vi "M-686 Stage Engine.vi"(0 "Notifier Name":string, 11 "COM Port":string[](array[string])) -> ()   [LabVIEW 2016]
uses:
  Stages Controls/Stage Notifier Element.ctl
  Stages Controls/Stage Actions.ctl
  Stages Controls/Stage Status.ctl
  <vilib>/Instr/_visa.llb/VISA Configure Serial Port (Instr).vi
panel:
  in  "Servo On/Off":bool
  in  "Quit":bool
  in  "Halt":bool
  in  "Home":bool
  in  "Get Position":bool
  in  "Y Position (µm)":dbl format="%#_4g"
  in  "X Position (µm)":dbl format="%#_4g"
  in  "XY Step Size (µm)":dbl format="%#_4g"
  in  "Up":bool
  in  "Down":bool
  in  "Left":bool
  in  "Right":bool
  in  "ReInitialize":bool
  in  "Error":bool
  # "(1) COM Port\n(2) Axis Name\n(3) Axis Name"
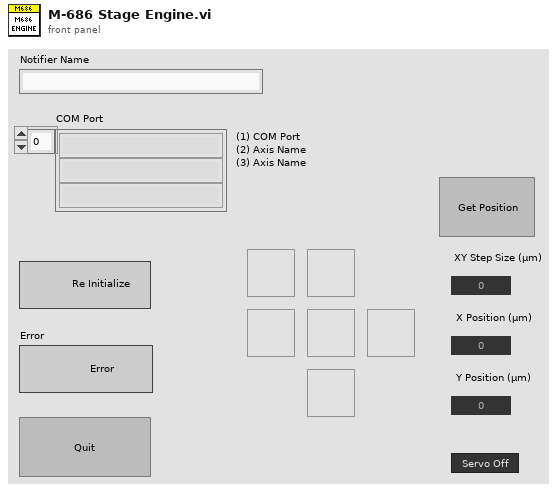
[diagram p1: front panel]
types:
  T1 = typedef "Stage Notifier Element.ctl" = cluster{"Action":T2, "Axis":bool[], "Setpoint":dbl[], "Velocity":dbl, "Cmd Recvd?":bool, "Position":dbl[], "Status":T3, "Misc":variant, "Servo On?":bool}
  T2 = typedef "Stage Actions.ctl" = enum16{"Get Position", "SERVO OFF", "SERVO ON", "SERVO ON/OFF", "MVR", "MOVE", "HALT", "ONTARGET", "ERROR", "REFERENCE", "INIT", "VELOCITY", "STATUS", "EXIT", "HOME", "ZEROPOS", "NANOPOS", "ANALOG", "QUIT"}
  T3 = typedef "Stage Status.ctl" = enum16{"Error", "Abort", "Busy", "On Target"}
  T4 = enum32{"Invalid", "Standard", "Closed", "Hidden", "Minimized", "Maximized"}
  T5 = enum8{"Enabled", "Disabled", "Disabled and Grayed Out"}
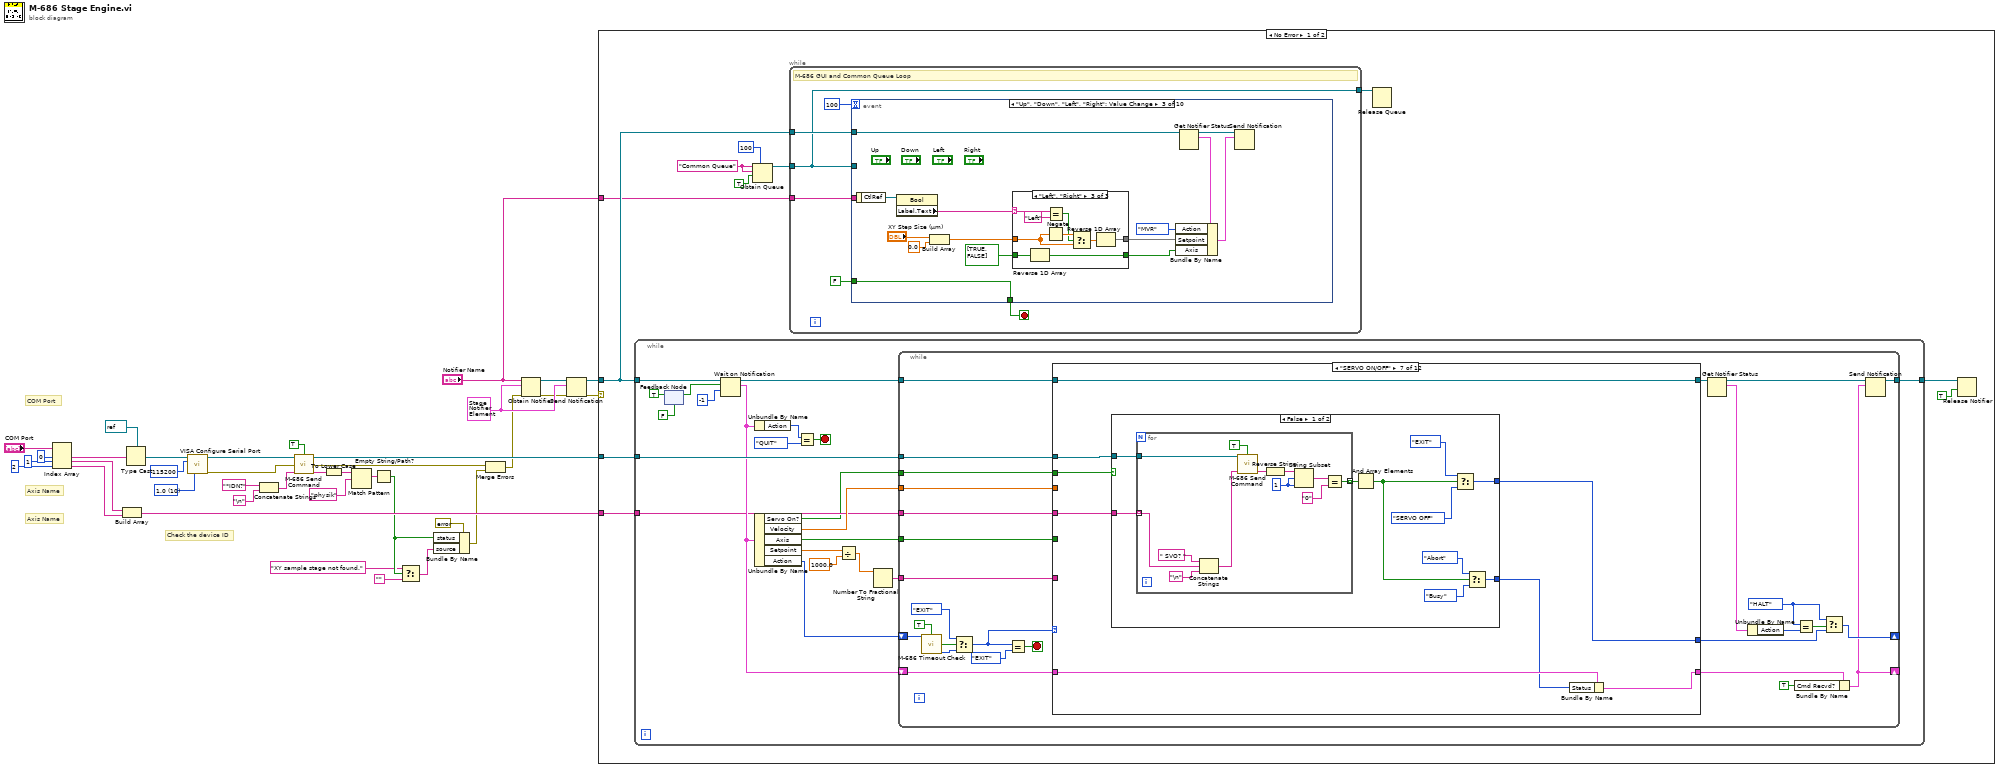
[diagram p0: block diagram]
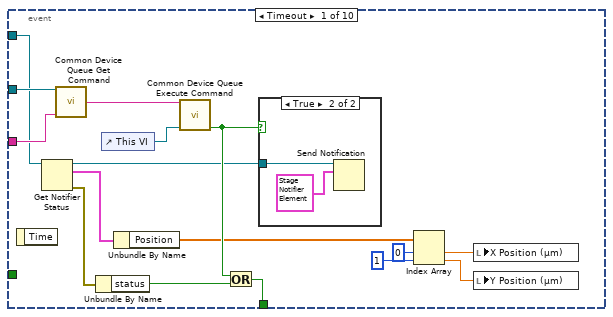
[diagram p2: hidden frame]
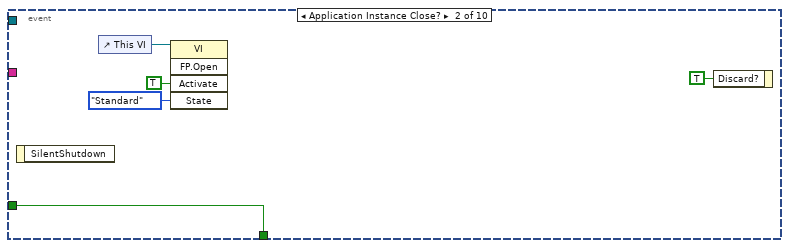
[diagram p4: hidden frame]
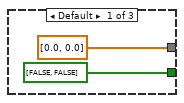
[diagram p5: hidden frame]
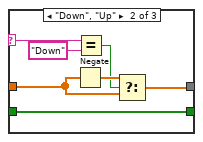
[diagram p6: hidden frame]
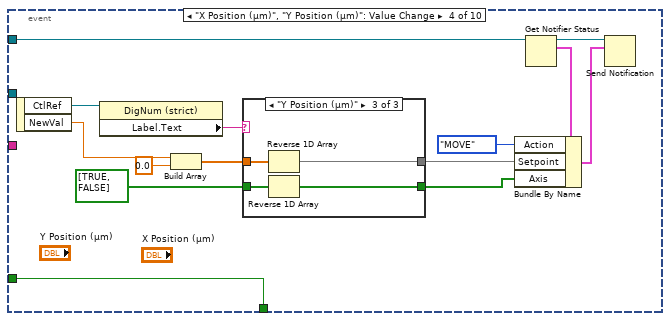
[diagram p7: hidden frame]
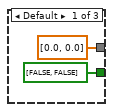
[diagram p8: hidden frame]
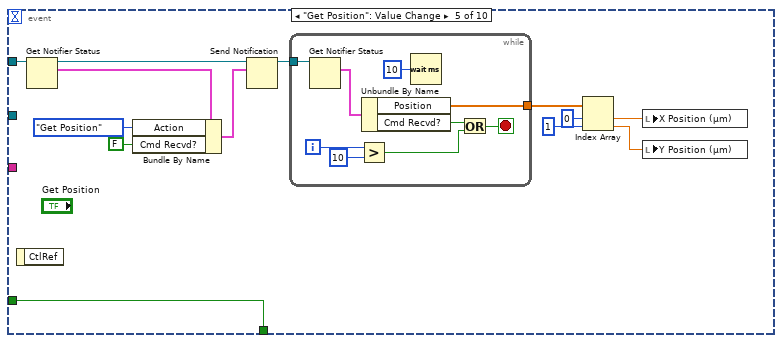
[diagram p10: hidden frame]
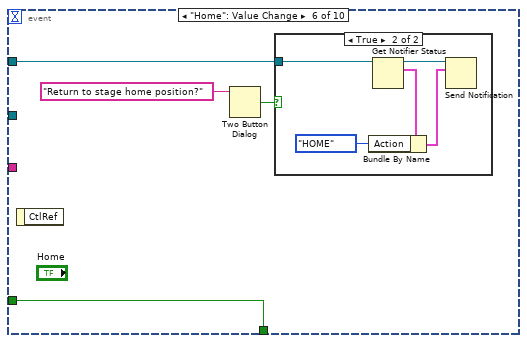
[diagram p11: hidden frame]
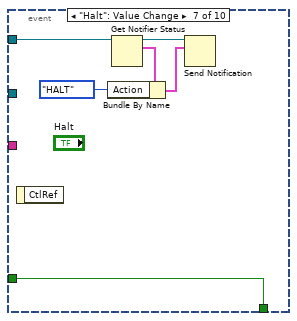
[diagram p13: hidden frame]
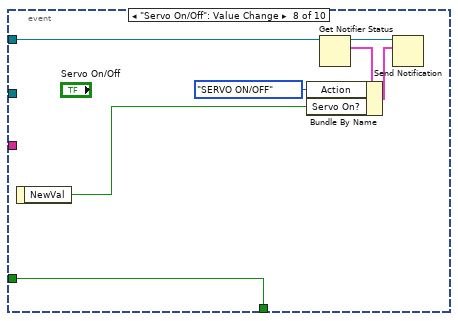
[diagram p14: hidden frame]
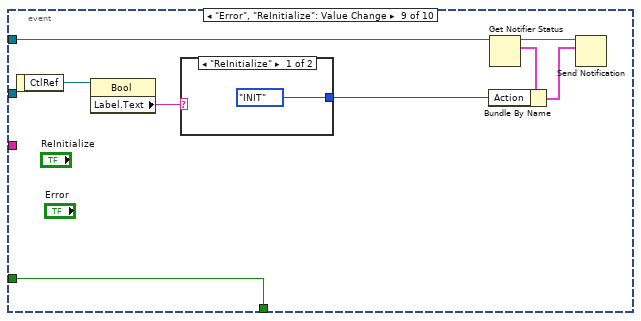
[diagram p15: hidden frame]
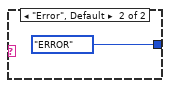
[diagram p16: hidden frame]
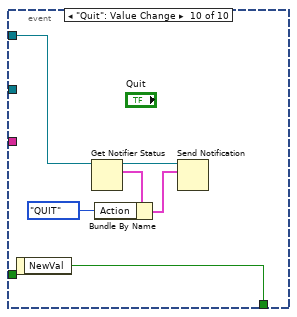
[diagram p17: hidden frame]
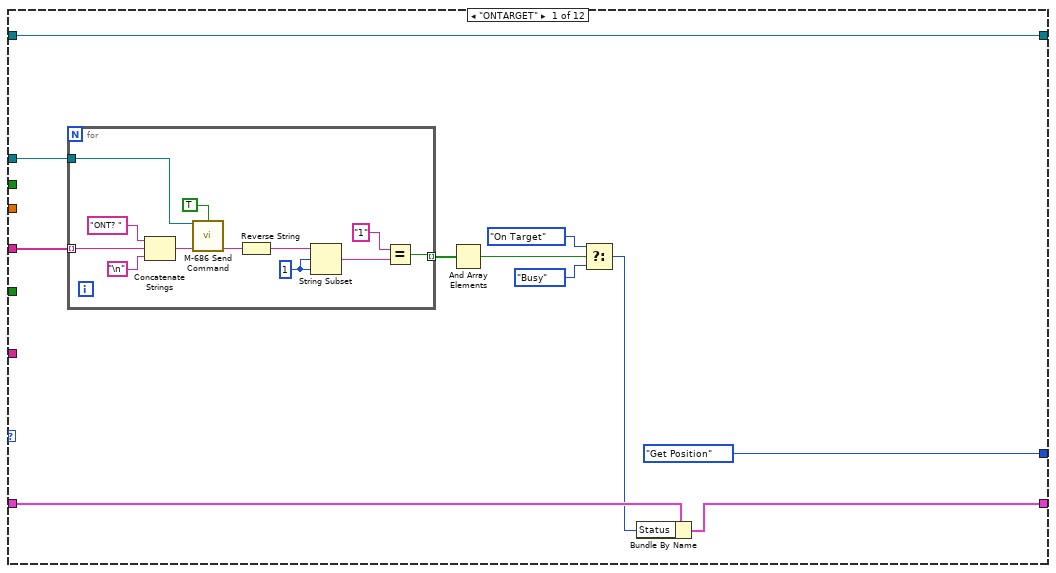
[diagram p18: hidden frame]
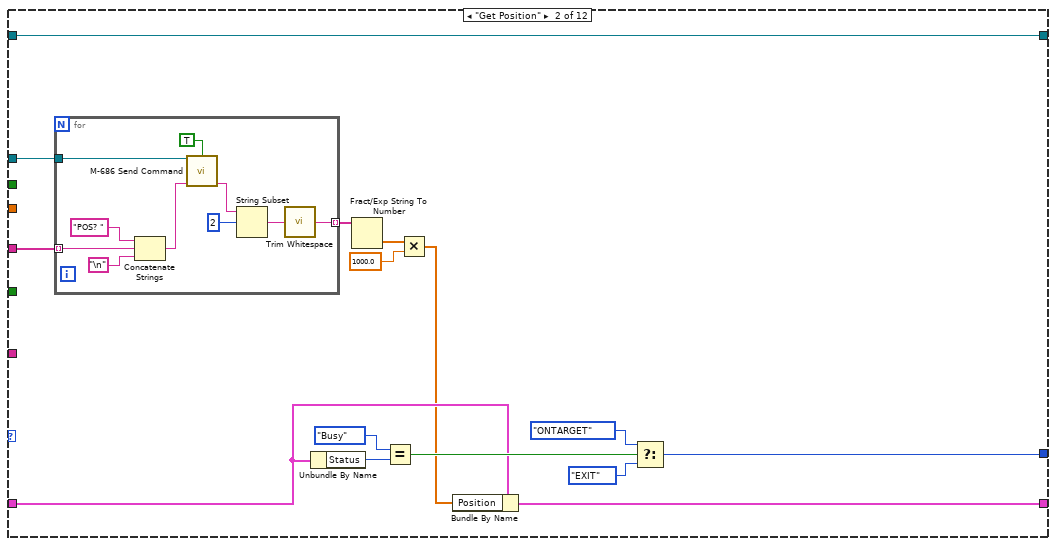
[diagram p19: hidden frame]
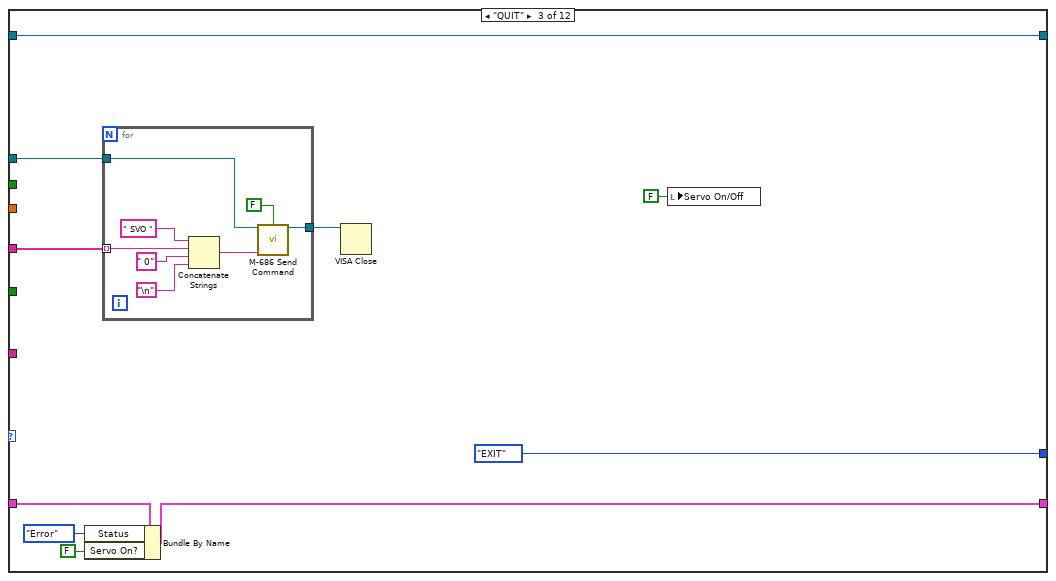
[diagram p20: hidden frame]
diagram:
  w21 = u16 10 items=["1.0"=10, "1.5"=15, "2.0"=20] ("stop bits (10: 1 bit)")
  w32 = T1 {"Action"=enum."INIT", "Axis"=[], "Setpoint"=[], "Velocity"=0.5, "Cmd Recvd?"=FALSE, "Position"=[], "Status"=enum."Busy", "Misc"=variant, "Servo On?"=FALSE} ("Stage Status")
  # "Check the device ID"
  # "Axis Name"
  # "Axis Name"
  # "COM Port"
  n1 = Index Array(array="COM Port", index #1=0 ("index"), index #2=1 ("index"), index #3=2 ("index")) -> (element #1=w36:string, element #2=w25:string, element #3=w24:string)
  n2 = Build Array(w25, w24) -> (w23:string[])
  n3 = Type Cast(type=refnum<visa-resource-name> refnum ("reference out"), x=w36) -> (*(type *) &x=w20:refnum<visa-resource-name>)
  n4 = call-poly "VISA Configure Serial Port"("VISA resource name"=w20, "baud rate (9600)"=u32 115200, "stop bits (10: 1 bit)"=w21) -> ("VISA resource name out"=w19:refnum<visa-resource-name>, "error out"=w18:errorcluster)  [unwired: 11 in]
  n5 = Concatenate Strings("*IDN?" ("string"), "\n") -> (w16:string)
  n6 = call "M-686 Send Command.vi"("VISA Ref"=w19, "Wait for Reply?"=TRUE, "Error In"=w18, "Command"=w16) -> ("VISA Ref Out"=w17:refnum<visa-resource-name>, "Error Out"=w7:errorcluster, "Response"=w9:string)  [unwired: 9 in]
  n7 = To Lower Case(string=w9) -> (all lower case string=w12:string)
  n8 = Match Pattern(string=w12, regular expression="physik" ("string")) -> (match substring=w11:string)  [unwired: 1 in, 3 out]
  n9 = Empty String/Path?(string/path=w11) -> (empty?=w4:bool)
  n10 = Select(t="XY sample stage not found." ("string"), s=w4, f="") -> (s? t:f=w3:string)
  n11 = Bundle By Name(cluster=errorcluster {"status"=FALSE, "code"=0, "source"=""} ("Error Out"), "status"=w4, "source"=w3) -> (w5:errorcluster)
  n12 = Merge Errors(w7, w5) -> (w6:errorcluster)
  n13 = Obtain Notifier(name (unnamed)="Notifier Name", notification data type=w32, error in (no error)=w6) -> (notifier out=w33:refnum<notifier>, error out=w31:errorcluster)  [unwired: 1 in, 1 out]
  n14 = Send Notification(notification=w32, notifier=w33, error in (no error)=w31) -> (notifier out=w30:refnum<notifier>, error out=w29:errorcluster)
  n15 = case shown="No Error" w29 {
    selector: w29 -> [_ w573]
    tunnel: w17 -> [w48 w574]
    tunnel: w30 -> [w41 w575]
    tunnel: "Notifier Name" -> [w40 _]
    tunnel: w23 -> [w38 _]
    frame No Error {
      w44 = "Common Queue" ("Unique Notifier Name")
      n16 = while {
        tunnel: w41 -> [w210]
        tunnel: w48 -> [w202]
        tunnel: [w199] -> w47
        tunnel: w38 -> [w195]
        stop <- w212 stop-if-true
        n17 = feedback-in #1(TRUE) -> ()
        n18 = feedback #1(FALSE) -> (w196:bool)
        n19 = Wait on Notification(notifier=w210, ignore previous (F)=w196, timeout in ms (-1)=-1) -> (notifier out=w201:refnum<notifier>, notification=w200:T1)  [unwired: 1 in, 2 out]
        n20 = Unbundle By Name(w200) -> ("Action"=w209:T2)
        n21 = Unbundle By Name(w200) -> ("Servo On?"=w192:bool, "Velocity"=w206:dbl, "Axis"=w205:bool[], "Setpoint"=w204:dbl[], "Action"=w194:T2)
        n22 = Equal?(x=w209, y=Stage_Actions."QUIT") -> (x = y?=w212:bool)
        n23 = Divide(x=w204, y=1000.0) -> (x/y=w193:dbl[])
        n24 = Number To Fractional String(number=w193) -> (F-format string=w207:string[])  [unwired: 3 in]
        n25 = while {
          tunnel: w195 -> [w240]
          shift-right: [w233] -> _
          shift-left: w194 -> [w230]
          tunnel: w205 -> [w237]
          tunnel: w206 -> [w236]
          tunnel: w207 -> [w238]
          shift-right: [w216] -> _
          shift-left: w200 -> [w235]
          tunnel: w202 -> [w239]
          tunnel: w201 -> [w215]
          tunnel: [w219] -> w199
          tunnel: w192 -> [w213]
          stop <- w231 stop-if-true
          w222 = Stage_Actions."HALT" ("Action")
          n26 = call "M-686 Timeout Check.vi"("Action"=w230, "User Input?"=TRUE) -> ("Timeout?"=w229:bool, "Action (Dup)"=w227:T2)  [unwired: 12 in]
          n27 = Select(t=Stage_Actions."EXIT" ("y"), s=w229, f=w227) -> (s? t:f=w226:T2)
          n28 = Equal?(x=w226, y=Stage_Actions."EXIT") -> (x = y?=w231:bool)
          n29 = case shown="\"SERVO ON/OFF\"" w226 {
            selector: w226 -> [_ _ _ _ _ _ _ _ _ _ _ w531]
            tunnel: w240 -> [w249 w277 w297 _ _ w345 w381 w434 w464 w482 w516 w543]
            tunnel: w239 -> [w251 w278 w298 _ w314 w336 w382 w435 w465 w481 w511 w537]
            tunnel: w238 -> [_ _ _ _ _ _ _ _ _ _ _ w534]
            tunnel: w237 -> [_ _ _ _ _ _ _ _ _ _ _ w525]
            tunnel: w236 -> [_ _ _ _ _ _ _ _ _ _ _ w542]
            tunnel: [Stage_Actions."Get Position" ("Action") w275 Stage_Actions."EXIT" ("Action") Stage_Actions."EXIT" ("Action") w324 w344 w380 w433 Stage_Actions."EXIT" ("Action") w477 Stage_Actions."EXIT" ("Action") Stage_Actions."ONTARGET" ("Action")] -> w234
            tunnel: w235 -> [w244 w272 w295 w309 w322 w346 w378 w431 w460 w475 w513 w539]
            tunnel: [w242 w270 w293 w309 w323 w347 w377 w429 w459 w474 w512 w538] -> w218
            tunnel: w215 -> [w241 w264 w289 w307 w310 w330 w379 w432 w462 w473 w510 w523]
            tunnel: [w241 w264 w289 w307 w310 w330 w379 w432 w462 w473 w510 w523] -> w214
            tunnel: w213 -> [_ _ _ _ _ _ w383 _ _ _ _ _]
            frame "ONTARGET" {
              n30 = for {
                tunnel: [w261] -> w250 mode=indexing
                tunnel: w249 -> [w256] mode=indexing
                tunnel: w251 -> [w253]
                w257 = 1 ("length (rest)")
                n31 = Concatenate Strings("ONT? " ("string"), w256, "\n") -> (w255:string)
                n32 = call "M-686 Send Command.vi"("VISA Ref"=w253, "Wait for Reply?"=TRUE, "Command"=w255) -> ("Response"=w252:string)  [unwired: 10 in, 2 out]
                n33 = Reverse String(1:w252) -> (0:w258:string)
                n34 = String Subset(string=w258, offset (0)=w257, length (rest)=w257) -> (substring=w263:string)
                n35 = Equal?(x="1", y=w263) -> (x = y?=w261:bool)
              }
              n36 = And Array Elements(Boolean array=w250) -> (logical AND=w245:bool)
              n37 = Select(t=Stage_Status."On Target" ("Status"), s=w245, f=Stage_Status."Busy" ("Status")) -> (s? t:f=w243:T3)
              n38 = Bundle By Name(cluster=w244, "Status"=w243) -> (w242:T1)
            }
            frame "Get Position" {
              n39 = for {
                tunnel: [w288] -> w276 mode=indexing
                tunnel: w277 -> [w283] mode=indexing
                tunnel: w278 -> [w282]
                n40 = Concatenate Strings("POS? " ("string"), w283, "\n") -> (w281:string)
                n41 = call "M-686 Send Command.vi"("VISA Ref"=w282, "Wait for Reply?"=TRUE, "Command"=w281) -> ("Response"=w279:string)  [unwired: 10 in, 2 out]
                n42 = String Subset(string=w279, offset (0)=2) -> (substring=w284:string)  [unwired: 1 in]
                n43 = call <vilib>:"Trim Whitespace.vi"("string"=w284) -> ("trimmed string"=w288:string)  [unwired: 1 in]
              }
              n44 = Unbundle By Name(w272) -> ("Status"=w271:T3)
              n45 = Fract/Exp String To Number(string=w276) -> (number=w269:dbl[])  [unwired: 3 in, 1 out]
              n46 = Equal?(x=Stage_Status."Busy", y=w271) -> (x = y?=w273:bool)
              n47 = Multiply(x=w269, y=1000.0) -> (x*y=w266:dbl[])
              n48 = Bundle By Name(cluster=w272, "Position"=w266) -> (w270:T1)
              n49 = Select(t=Stage_Actions."ONTARGET" ("Action"), s=w273, f=Stage_Actions."EXIT" ("Action")) -> (s? t:f=w275:T2)
            }
            frame "QUIT" {
              n50 = Bundle By Name(cluster=w295, "Status"=Stage_Status."Error", "Servo On?"=FALSE) -> (w293:T1)
              n51 = for {
                tunnel: w298 -> [w300]
                tunnel: w297 -> [w303] mode=indexing
                tunnel: [w299] -> w292
                n52 = Concatenate Strings(" SVO " ("string"), w303, " 0" ("string"), "\n") -> (w302:string)
                n53 = call "M-686 Send Command.vi"("VISA Ref"=w300, "Wait for Reply?"=FALSE, "Command"=w302) -> ("VISA Ref Out"=w299:refnum<visa-resource-name>)  [unwired: 10 in, 2 out]
              }
              n54 = VISA Close(VISA resource name=w292) -> ()  [unwired: 1 in, 1 out]
              n55 = local write "Servo On/Off"(FALSE ("Servo On/Off")) -> ()
            }
            frame "EXIT", Default {
            }
            frame "ERROR" {
              n56 = Concatenate Strings(" ERR?" ("string"), "\n") -> (w312:string)
              n57 = call "M-686 Send Command.vi"("VISA Ref"=w314, "Wait for Reply?"=TRUE, "Command"=w312) -> ("Response"=w311:string)  [unwired: 10 in, 2 out]
              n58 = Reverse String(1:w311) -> (0:w319:string)
              n59 = String Subset(string=w319, offset (0)=1) -> (substring=w321:string)  [unwired: 1 in]
              n60 = Equal?(x=w321, y="0") -> (x = y?=w315:bool)
              n61 = Select(t=Stage_Status."Busy" ("Status"), s=w315, f=Stage_Status."Error" ("Status")) -> (s? t:f=w327:T3)
              n62 = Bundle By Name(cluster=w322, "Status"=w327) -> (w323:T1)
              n63 = Select(t=Stage_Actions."ONTARGET" ("Action"), s=w315, f=Stage_Actions."ERROR") -> (s? t:f=w324:T2)
            }
            frame "INIT" {
              n64 = Concatenate Strings(" ERR?" ("string"), "\n") -> (w333:string)
              n65 = call "M-686 Send Command.vi"("VISA Ref"=w336, "Wait for Reply?"=TRUE, "Command"=w333) -> ("VISA Ref Out"=w335:refnum<visa-resource-name>, "Response"=w332:string)  [unwired: 10 in, 1 out]
              n66 = Reverse String(1:w332) -> (0:w342:string)
              n67 = String Subset(string=w342, offset (0)=1) -> (substring=w340:string)  [unwired: 1 in]
              n68 = Equal?(x=w340, y="0") -> (x = y?=w337:bool)
              n69 = case shown="True" w337 {
                tunnel: w345 -> [_ w357]
                tunnel: [Stage_Actions."INIT" ("Action") w355] -> w344
                tunnel: w335 -> [_ w353]
                tunnel: [w349 w351] -> w331
                frame False {
                  w349 = FALSE
                  n70 = local write "Servo On/Off"(w349) -> ()
                }
                frame True {
                  n71 = for {
                    tunnel: w357 -> [w371] mode=indexing
                    tunnel: w353 -> [w364]
                    tunnel: [w366] -> w352 mode=indexing
                    w370 = 1 ("length (rest)")
                    n72 = Concatenate Strings(" SVO " ("string"), w371, " 1" ("string"), "\n") -> (w363:string)
                    n73 = Concatenate Strings(" SVO? " ("string"), w371, "\n") -> (w360:string)
                    n74 = call "M-686 Send Command.vi"("VISA Ref"=w364, "Wait for Reply?"=FALSE, "Command"=w363) -> ("VISA Ref Out"=w361:refnum<visa-resource-name>)  [unwired: 10 in, 2 out]
                    n75 = call "M-686 Send Command.vi"("VISA Ref"=w361, "Wait for Reply?"=TRUE, "Command"=w360) -> ("Response"=w358:string)  [unwired: 10 in, 2 out]
                    n76 = Reverse String(1:w358) -> (0:w369:string)
                    n77 = String Subset(string=w369, offset (0)=w370, length (rest)=w370) -> (substring=w368:string)
                    n78 = Equal?(x=w368, y="1") -> (x = y?=w366:bool)
                  }
                  n79 = And Array Elements(Boolean array=w352) -> (logical AND=w351:bool)
                  n80 = local write "Servo On/Off"(w351) -> ()
                  n81 = Select(t=Stage_Actions."REFERENCE" ("Action"), s=w351, f=Stage_Actions."INIT" ("Action")) -> (s? t:f=w355:T2)
                }
              }
              n82 = Bundle By Name(cluster=w346, "Status"=Stage_Status."Busy", "Servo On?"=w331) -> (w347:T1)
            }
            frame "SERVO ON/OFF" {
              n83 = case shown="False" w383 {
                tunnel: w381 -> [w389 w415]
                tunnel: [w388 w410] -> w380
                tunnel: w382 -> [w390 w414]
                tunnel: [w384 w406] -> w376
                frame False {
                  n84 = for {
                    tunnel: w389 -> [w403] mode=indexing
                    tunnel: w390 -> [w394]
                    tunnel: [w398] -> w393 mode=indexing
                    w402 = 1 ("length (rest)")
                    n85 = Concatenate Strings(" SVO? " ("string"), w403, "\n") -> (w397:string)
                    n86 = call "M-686 Send Command.vi"("VISA Ref"=w394, "Wait for Reply?"=TRUE, "Command"=w397) -> ("Response"=w395:string)  [unwired: 10 in, 2 out]
                    n87 = Reverse String(1:w395) -> (0:w401:string)
                    n88 = String Subset(string=w401, offset (0)=w402, length (rest)=w402) -> (substring=w400:string)
                    n89 = Equal?(x=w400, y="0") -> (x = y?=w398:bool)
                  }
                  n90 = And Array Elements(Boolean array=w393) -> (logical AND=w385:bool)
                  n91 = Select(t=Stage_Actions."EXIT" ("Action"), s=w385, f=Stage_Actions."SERVO OFF") -> (s? t:f=w388:T2)
                  n92 = Select(t=Stage_Status."Abort", s=w385, f=Stage_Status."Busy" ("Status")) -> (s? t:f=w384:T3)
                }
                frame True {
                  n93 = for {
                    tunnel: w415 -> [w425] mode=indexing
                    tunnel: w414 -> [w416]
                    tunnel: [w420] -> w413 mode=indexing
                    w424 = 1 ("length (rest)")
                    n94 = Concatenate Strings(" SVO? " ("string"), w425, "\n") -> (w419:string)
                    n95 = call "M-686 Send Command.vi"("VISA Ref"=w416, "Wait for Reply?"=TRUE, "Command"=w419) -> ("Response"=w417:string)  [unwired: 10 in, 2 out]
                    n96 = Reverse String(1:w417) -> (0:w423:string)
                    n97 = String Subset(string=w423, offset (0)=w424, length (rest)=w424) -> (substring=w422:string)
                    n98 = Equal?(x=w422, y="1") -> (x = y?=w420:bool)
                  }
                  n99 = And Array Elements(Boolean array=w413) -> (logical AND=w409:bool)
                  n100 = Select(t=Stage_Actions."EXIT" ("Action"), s=w409, f=Stage_Actions."SERVO ON") -> (s? t:f=w410:T2)
                  n101 = Select(t=Stage_Status."On Target", s=w409, f=Stage_Status."Busy" ("Status")) -> (s? t:f=w406:T3)
                }
              }
              n102 = Bundle By Name(cluster=w378, "Status"=w376) -> (w377:T1)
            }
            frame "SERVO ON" {
              w428 = T5."Enabled" ("Disabled")
              n103 = for {
                tunnel: w434 -> [w453] mode=indexing
                tunnel: w435 -> [w446]
                tunnel: [w448] -> w436 mode=indexing
                w452 = 1 ("length (rest)")
                n104 = Concatenate Strings(" SVO " ("string"), w453, " 1" ("string"), "\n") -> (w445:string)
                n105 = Concatenate Strings(" SVO? " ("string"), w453, "\n") -> (w442:string)
                n106 = call "M-686 Send Command.vi"("VISA Ref"=w446, "Wait for Reply?"=FALSE, "Command"=w445) -> ("VISA Ref Out"=w443:refnum<visa-resource-name>)  [unwired: 10 in, 2 out]
                n107 = call "M-686 Send Command.vi"("VISA Ref"=w443, "Wait for Reply?"=TRUE, "Command"=w442) -> ("Response"=w440:string)  [unwired: 10 in, 2 out]
                n108 = Reverse String(1:w440) -> (0:w451:string)
                n109 = String Subset(string=w451, offset (0)=w452, length (rest)=w452) -> (substring=w450:string)
                n110 = Equal?(x=w450, y="1") -> (x = y?=w448:bool)
              }
              n111 = Bundle By Name(cluster=w431, "Status"=Stage_Status."Busy") -> (w429:T1)
              n112 = And Array Elements(Boolean array=w436) -> (logical AND=w437:bool)
              n113 = Select(t=Stage_Actions."Get Position" ("Action"), s=w437, f=Stage_Actions."SERVO ON" ("Action")) -> (s? t:f=w433:T2)
              n114 = property on="Down" class="Bool"("DisabledEnum"=w428) -> ()  [unwired: 2 in, 2 out]
              n115 = property on="Up" class="Bool"("DisabledEnum"=w428) -> ()  [unwired: 2 in, 2 out]
              n116 = property on="Y Position (µm)" class="DigNum (strict)"("DisabledEnum"=w428) -> ()  [unwired: 2 in, 2 out]
              n117 = property on="Right" class="Bool"("DisabledEnum"=w428) -> ()  [unwired: 2 in, 2 out]
              n118 = property on="Left" class="Bool"("DisabledEnum"=w428) -> ()  [unwired: 2 in, 2 out]
              n119 = property on="X Position (µm)" class="DigNum (strict)"("DisabledEnum"=w428) -> ()  [unwired: 2 in, 2 out]
            }
            frame "SERVO OFF" {
              w458 = T5."Disabled and Grayed Out" ("Disabled")
              n120 = for {
                tunnel: w465 -> [w466]
                tunnel: w464 -> [w469] mode=indexing
                n121 = Concatenate Strings(" SVO " ("string"), w469, " 0" ("string"), "\n") -> (w468:string)
                n122 = call "M-686 Send Command.vi"("VISA Ref"=w466, "Wait for Reply?"=FALSE, "Command"=w468) -> ()  [unwired: 10 in, 3 out]
              }
              n123 = Bundle By Name(cluster=w460, "Status"=Stage_Status."Abort") -> (w459:T1)
              n124 = property on="X Position (µm)" class="DigNum (strict)"("DisabledEnum"=w458) -> ()  [unwired: 2 in, 2 out]
              n125 = property on="Y Position (µm)" class="DigNum (strict)"("DisabledEnum"=w458) -> ()  [unwired: 2 in, 2 out]
              n126 = property on="Down" class="Bool"("DisabledEnum"=w458) -> ()  [unwired: 2 in, 2 out]
              n127 = property on="Right" class="Bool"("DisabledEnum"=w458) -> ()  [unwired: 2 in, 2 out]
              n128 = property on="Left" class="Bool"("DisabledEnum"=w458) -> ()  [unwired: 2 in, 2 out]
              n129 = property on="Up" class="Bool"("DisabledEnum"=w458) -> ()  [unwired: 2 in, 2 out]
            }
            frame "REFERENCE" {
              n130 = for {
                tunnel: w482 -> [w507] mode=indexing
                tunnel: w481 -> [w501]
                tunnel: [w500] -> w478
                tunnel: [w502] -> w480 mode=indexing
                w505 = 1 ("length (rest)")
                n131 = Concatenate Strings(" FRF? " ("string"), w507, "\n") -> (w499:string)
                n132 = call "M-686 Send Command.vi"("VISA Ref"=w501, "Wait for Reply?"=TRUE, "Command"=w499) -> ("VISA Ref Out"=w500:refnum<visa-resource-name>, "Response"=w498:string)  [unwired: 10 in, 1 out]
                n133 = Reverse String(1:w498) -> (0:w506:string)
                n134 = String Subset(string=w506, offset (0)=w505, length (rest)=w505) -> (substring=w503:string)
                n135 = Equal?(x=w503, y="1") -> (x = y?=w502:bool)
              }
              n136 = Bundle By Name(cluster=w475, "Status"=Stage_Status."Busy") -> (w474:T1)
              n137 = And Array Elements(Boolean array=w480) -> (logical AND=w479:bool)
              n138 = case shown="True" w479 {
                tunnel: w478 -> [w484 _]
                tunnel: [w483 Stage_Actions."ONTARGET" ("Action")] -> w477
                frame False {
                  n139 = Two Button Dialog(message="M686", 1:"Skip" ("F button name (\"Cancel\")"), 2:"Reference" ("T button name (\"OK\")")) -> (T button?=w488:bool)
                  n140 = case shown="True" w488 {
                    tunnel: [Stage_Actions."HALT" ("Action") Stage_Actions."ONTARGET" ("Action")] -> w483
                    tunnel: w484 -> [_ w492]
                    frame False {
                    }
                    frame True {
                      n141 = Concatenate Strings("FRF" ("string"), "\n") -> (w491:string)
                      n142 = call "M-686 Send Command.vi"("VISA Ref"=w492, "Wait for Reply?"=FALSE, "Command"=w491) -> ()  [unwired: 10 in, 3 out]
                    }
                  }
                }
                frame True {
                }
              }
            }
            frame "HALT" {
              n143 = for {
                tunnel: w516 -> [w520] mode=indexing
                tunnel: w511 -> [w518]
                n144 = Concatenate Strings(w520, " HLT" ("string"), "\n") -> (w519:string)
                n145 = call "M-686 Send Command.vi"("VISA Ref"=w518, "Wait for Reply?"=FALSE, "Command"=w519) -> ()  [unwired: 10 in, 3 out]
              }
              n146 = Bundle By Name(cluster=w513, "Status"=Stage_Status."Abort") -> (w512:T1)
            }
            frame "MVR", "MOVE", "HOME" {
              n147 = Bundle By Name(cluster=w539, "Status"=Stage_Status."Busy") -> (w538:T1)
              n148 = Equal?(x=Stage_Actions."MVR", y=w531) -> (x = y?=w524:bool)
              n149 = Equal?(x=w531, y=Stage_Actions."HOME") -> (x = y?=w535:bool)
              n150 = Not(x=w535) -> (.not. x?=w530:bool)
              n151 = Select(t="MVR ", s=w524, f="MOV ") -> (s? t:f=w526:string)
              n152 = Select(t=w534, s=w530, f=string[] ["12.5", "12.5"]) -> (s? t:f=w533:string[])
              n153 = for {
                tunnel: w543 -> [w549] mode=indexing
                tunnel: w533 -> [w548] mode=indexing
                tunnel: w525 -> [w547] mode=indexing
                tunnel: w542 -> [w546]
                tunnel: w537 -> [w545]
                tunnel: w526 -> [w544]
                n154 = case shown="True" w547 {
                  tunnel: w549 -> [_ w557]
                  tunnel: w548 -> [_ w558]
                  tunnel: w545 -> [_ w551]
                  tunnel: w546 -> [_ w556]
                  tunnel: w544 -> [_ w550]
                  frame False {
                  }
                  frame True {
                    n155 = Equal To 0?(x=w556) -> (x = 0?=w555:bool)
                    n156 = call <vilib>:"Space Constant.vi"() -> ("String"=w559:string)
                    n157 = case shown="False" w555 {
                      tunnel: w557 -> [w567 _]
                      tunnel: w556 -> [w564 _]
                      tunnel: [w566 ""] -> w554
                      frame False {
                        n158 = Number To Fractional String(number=w564) -> (F-format string=w565:string)  [unwired: 3 in]
                        n159 = call <vilib>:"Space Constant.vi"() -> ("String"=w570:string)
                        n160 = Concatenate Strings("VEL ", w567, w570, w565, "\n") -> (w566:string)
                      }
                      frame True {
                      }
                    }
                    n161 = Concatenate Strings(w550, w557, w559, w558, "\n") -> (w553:string)
                    n162 = Build Array(w554, w553) -> (w552:string[])
                    n163 = for {
                      tunnel: w552 -> [w563] mode=indexing
                      tunnel: w551 -> [w561]
                      n164 = call "M-686 Send Command.vi"("VISA Ref"=w561, "Wait for Reply?"=FALSE, "Command"=w563) -> ()  [unwired: 10 in, 3 out]
                    }
                  }
                }
              }
            }
          }
          n165 = Get Notifier Status(notifier=w214) -> (notifier out=w220:refnum<notifier>, current notification=w221:T1)  [unwired: 1 in, 3 out]
          n166 = Unbundle By Name(w221) -> ("Action"=w223:T2)
          n167 = Bundle By Name(cluster=w218, "Cmd Recvd?"=TRUE) -> (w216:T1)
          n168 = Equal?(x=w222, y=w223) -> (x = y?=w224:bool)
          n169 = Select(t=w222, s=w224, f=w234) -> (s? t:f=w233:T2)
          n170 = Send Notification(notification=w216, notifier=w220) -> (notifier out=w219:refnum<notifier>)  [unwired: 1 in, 1 out]
        }
      }
      n171 = Obtain Queue(max queue size (-1, unlimited)=100, name (unnamed)=w44, element data type=w44, create if not found? (T)=TRUE) -> (queue out=w45:refnum<queue>)  [unwired: 1 in, 2 out]
      n172 = while {
        tunnel: w45 -> [w49]
        tunnel: w40 -> [w52]
        tunnel: w41 -> [w53]
        tunnel: [w49] -> w39
        stop <- w51 stop-if-true
        # "M-686 GUI and Common Queue Loop"
        n173 = event shown="[2] \"Up\", \"Down\", \"Left\", \"Right\": Value Change" {
          selector: _ -> [_ _ _ _ _ _ _ _ _ _]
          dyn-events: _ -> [_ _ _ _ _ _ _ _ _ _]
          timeout: 100 -> [_ _ _ _ _ _ _ _ _ _]
          tunnel: w49 -> [w64 _ _ _ _ _ _ _ _ _]
          tunnel: w53 -> [w61 _ w84 w116 w143 w154 w167 w171 w180 w191]
          tunnel: w52 -> [w63 _ _ _ _ _ _ _ _ _]
          tunnel: [w62 w77 w87 w123 w144 w156 w168 w169 w183 w187] -> w51
          tunnel: FALSE -> [_ w77 w87 w123 w144 w156 w168 w169 w183 _]
          event Timeout {
            n174 = event-data() -> ()  [unwired: 1 in, 1 out]
            n175 = Get Notifier Status(notifier=w61) -> (notifier out=w65:refnum<notifier>, current notification=w60:T1, error out=w70:errorcluster)  [unwired: 1 in, 2 out]
            n176 = call "Common Device Queue Get Command.vi"("Common Queue"=w64, "Notifier Name"=w63) -> ("Command"=w69:string)  [unwired: 12 in, 1 out]
            n177 = Unbundle By Name(w70) -> ("status"=w67:bool)
            n178 = control-ref of="This VI"() -> (w68:refnum<vi>)
            n179 = Unbundle By Name(w60) -> ("Position"=w55:dbl[])
            n180 = call "Common Device Queue Execute Command.vi"("Common Command"=w69, "VI Refnum"=w68) -> ("Quit?"=w66:bool)  [unwired: 12 in, 1 out]
            n181 = Or(x=w66, y=w67) -> (x .or. y?=w62:bool)
            n182 = case shown="True" w66 {
              tunnel: w65 -> [_ w72]
              frame False {
              }
              frame True {
                n183 = Send Notification(notification=T1 {"Action"=enum."QUIT", "Axis"=[], "Setpoint"=[], "Velocity"=0.5, "Cmd Recvd?"=FALSE, "Position"=[], "Status"=enum."Error", "Misc"=variant, "Servo On?"=FALSE} ("Stage Status"), notifier=w72) -> ()  [unwired: 1 in, 2 out]
              }
            }
            n184 = Index Array(array=w55, index #1=0 ("index"), index #2=1 ("index")) -> (element #1=w59:dbl, element #2=w58:dbl)
            n185 = local write "X Position (µm)"(w59) -> ()
            n186 = local write "Y Position (µm)"(w58) -> ()
          }
          event Application Instance Close? {
            n187 = event-data() -> ()  [unwired: 1 in, 1 out]
            n188 = control-ref of="This VI"() -> (w74:refnum<vi>)
            n189 = invoke class="VI" method="FP.Open"(reference=w74, "Activate"=TRUE ("Activate?"), "State"=T4."Standard") -> ()  [unwired: 2 in, 5 out]
            n190 = event-data("Discard?"=TRUE) -> ()  [unwired: 1 in, 1 out]
          }
          event "Up", "Down", "Left", "Right": Value Change {
            n191 = event-data() -> ("CtlRef"=w86:refnum<vi>)  [unwired: 1 in]
            n192 = property class="Bool"(reference=w86) -> ("Label.Text"=w91:string)  [unwired: 1 in, 2 out]
            n193 = Build Array("XY Step Size (µm)", 0.0 ("element")) -> (w89:dbl[])
            n194 = case shown="\"Left\", \"Right\"" w91 {
              selector: w91 -> [_ w100 w106]
              tunnel: w89 -> [_ w97 w105]
              tunnel: bool[] [TRUE, FALSE] -> [_ w94 w103]
              tunnel: [dbl[] [0.0, 0.0] w96 w102] -> w82
              tunnel: [bool[] [FALSE, FALSE] w94 w101] -> w81
              frame Default {
              }
              frame "Down", "Up" {
                n195 = Negate(x=w97) -> (-x=w98:dbl[])
                n196 = Equal?(x=w100, y="Down") -> (x = y?=w95:bool)
                n197 = Select(t=w98, s=w95, f=w97) -> (s? t:f=w96:dbl[])
              }
              frame "Left", "Right" {
                n198 = Reverse 1D Array(array=w103) -> (reversed array=w101:bool[])
                n199 = Negate(x=w105) -> (-x=w108:dbl[])
                n200 = Equal?(x=w106, y="Left") -> (x = y?=w107:bool)
                n201 = Select(t=w108, s=w107, f=w105) -> (s? t:f=w104:dbl[])
                n202 = Reverse 1D Array(array=w104) -> (reversed array=w102:dbl[])
              }
            }
            n203 = Get Notifier Status(notifier=w84) -> (notifier out=w79:refnum<notifier>, current notification=w83:T1)  [unwired: 1 in, 3 out]
            n204 = Bundle By Name(cluster=w83, "Action"=Stage_Actions."MVR", "Setpoint"=w82, "Axis"=w81) -> (w78:T1)
            n205 = Send Notification(notification=w78, notifier=w79) -> ()  [unwired: 1 in, 2 out]
          }
          event "X Position (µm)", "Y Position (µm)": Value Change {
            n206 = event-data() -> ("CtlRef"=w118:refnum<vi>, "NewVal"=w117:dbl)  [unwired: 1 in]
            n207 = property class="DigNum (strict)"(reference=w118) -> ("Label.Text"=w121:string)  [unwired: 1 in, 2 out]
            n208 = Build Array(w117, 0.0 ("element")) -> (w122:dbl[])
            n209 = case shown="\"Y Position (µm)\"" w121 {
              tunnel: w122 -> [_ w127 w131]
              tunnel: bool[] [TRUE, FALSE] -> [_ w126 w130]
              tunnel: [dbl[] [0.0, 0.0] w127 w129] -> w113
              tunnel: [bool[] [FALSE, FALSE] w126 w128] -> w112
              frame Default {
              }
              frame "X Position (µm)" {
              }
              frame "Y Position (µm)" {
                n210 = Reverse 1D Array(array=w131) -> (reversed array=w129:dbl[])
                n211 = Reverse 1D Array(array=w130) -> (reversed array=w128:bool[])
              }
            }
            n212 = Get Notifier Status(notifier=w116) -> (notifier out=w115:refnum<notifier>, current notification=w114:T1)  [unwired: 1 in, 3 out]
            n213 = Bundle By Name(cluster=w114, "Action"=Stage_Actions."MOVE", "Setpoint"=w113, "Axis"=w112) -> (w110:T1)
            n214 = Send Notification(notification=w110, notifier=w115) -> ()  [unwired: 1 in, 2 out]
          }
          event "Get Position": Value Change {
            n215 = event-data() -> ()  [unwired: 1 in, 1 out]
            n216 = Get Notifier Status(notifier=w143) -> (notifier out=w142:refnum<notifier>, current notification=w141:T1)  [unwired: 1 in, 3 out]
            n217 = Bundle By Name(cluster=w141, "Action"=Stage_Actions."Get Position", "Cmd Recvd?"=FALSE) -> (w138:T1)
            n218 = Send Notification(notification=w138, notifier=w142) -> (notifier out=w137:refnum<notifier>)  [unwired: 1 in, 1 out]
            n219 = while {
              tunnel: w137 -> [w153]
              tunnel: [w145] -> w136
              i -> [w149]
              stop <- w146 stop-if-true
              n220 = Get Notifier Status(notifier=w153) -> (current notification=w152:T1)  [unwired: 1 in, 4 out]
              n221 = Greater?(x=w149, y=10) -> (0:w147:bool)
              n222 = Unbundle By Name(w152) -> ("Position"=w145:dbl[], "Cmd Recvd?"=w148:bool)
              n223 = Wait (ms)(milliseconds to wait=u32 10) -> ()  [unwired: 1 out]
              n224 = Or(x=w148, y=w147) -> (x .or. y?=w146:bool)
            }
            n225 = Index Array(array=w136, index #1=0 ("index"), index #2=1 ("index")) -> (element #1=w133:dbl, element #2=w132:dbl)
            n226 = local write "X Position (µm)"(w133) -> ()
            n227 = local write "Y Position (µm)"(w132) -> ()
          }
          event "Home": Value Change {
            n228 = event-data() -> ()  [unwired: 1 in, 1 out]
            n229 = Two Button Dialog(message="Return to stage home position?") -> (T button?=w155:bool)  [unwired: 2 in]
            n230 = case shown="True" w155 {
              tunnel: w154 -> [_ w162]
              frame False {
              }
              frame True {
                n231 = Get Notifier Status(notifier=w162) -> (notifier out=w161:refnum<notifier>, current notification=w160:T1)  [unwired: 1 in, 3 out]
                n232 = Bundle By Name(cluster=w160, "Action"=Stage_Actions."HOME") -> (w159:T1)
                n233 = Send Notification(notification=w159, notifier=w161) -> ()  [unwired: 1 in, 2 out]
              }
            }
          }
          event "Halt": Value Change {
            n234 = event-data() -> ()  [unwired: 1 in, 1 out]
            n235 = Get Notifier Status(notifier=w167) -> (notifier out=w166:refnum<notifier>, current notification=w165:T1)  [unwired: 1 in, 3 out]
            n236 = Bundle By Name(cluster=w165, "Action"=Stage_Actions."HALT") -> (w164:T1)
            n237 = Send Notification(notification=w164, notifier=w166) -> ()  [unwired: 1 in, 2 out]
          }
          event "Servo On/Off": Value Change {
            n238 = event-data() -> ("NewVal"=w170:bool)  [unwired: 1 in]
            n239 = Get Notifier Status(notifier=w171) -> (notifier out=w172:refnum<notifier>, current notification=w173:T1)  [unwired: 1 in, 3 out]
            n240 = Bundle By Name(cluster=w173, "Action"=Stage_Actions."SERVO ON/OFF", "Servo On?"=w170) -> (w174:T1)
            n241 = Send Notification(notification=w174, notifier=w172) -> ()  [unwired: 1 in, 2 out]
          }
          event "Error", "ReInitialize": Value Change {
            n242 = event-data() -> ("CtlRef"=w182:refnum<vi>)  [unwired: 1 in]
            n243 = property class="Bool"(reference=w182) -> ("Label.Text"=w181:string)  [unwired: 1 in, 2 out]
            n244 = case shown="\"ReInitialize\"" w181 {
              tunnel: [Stage_Actions."INIT" ("Action") Stage_Actions."ERROR" ("Action")] -> w176
              frame "ReInitialize" {
              }
              frame "Error", Default {
              }
            }
            n245 = Get Notifier Status(notifier=w180) -> (notifier out=w179:refnum<notifier>, current notification=w178:T1)  [unwired: 1 in, 3 out]
            n246 = Bundle By Name(cluster=w178, "Action"=w176) -> (w177:T1)
            n247 = Send Notification(notification=w177, notifier=w179) -> ()  [unwired: 1 in, 2 out]
          }
          event "Quit": Value Change {
            n248 = event-data() -> ("NewVal"=w187:bool)  [unwired: 1 in]
            n249 = Get Notifier Status(notifier=w191) -> (notifier out=w190:refnum<notifier>, current notification=w189:T1)  [unwired: 1 in, 3 out]
            n250 = Bundle By Name(cluster=w189, "Action"=Stage_Actions."QUIT") -> (w188:T1)
            n251 = Send Notification(notification=w188, notifier=w190) -> ()  [unwired: 1 in, 2 out]
          }
        }
      }
      n252 = Release Queue(queue=w39) -> ()  [unwired: 2 in, 3 out]
      n253 = Release Notifier(notifier=w47, force destroy? (F)=TRUE) -> ()  [unwired: 1 in, 3 out]
    }
    frame Error {
      n254 = VISA Close(VISA resource name=w574, error in (no error)=w573) -> (error out=w572:errorcluster)
      n255 = Release Notifier(notifier=w575, force destroy? (F)=TRUE, error in (no error)=w572) -> (error out=w580:errorcluster)  [unwired: 2 out]
      n256 = Unbundle By Name(w580) -> ("source"=w577:string)
      n257 = Concatenate Strings("M-686 (XY Sample Stage) Initialization Error", "\r", w577) -> (w576:string)
      n258 = One Button Dialog(message=w576) -> ()  [unwired: 1 in, 1 out]
    }
  }
